vi "NEO Swerve Drive.vi"(7 "Operation":T4, 9 "Drive Conditions":T3, 10 "Robot Velocities":T9, 11 "Motors In":T5 {"Steer Scaling" format="%.2f"; "Drive Scaling" format="%.2f"; "Pod Locations (ft)"."Right Back Position" format="%.2f"; "Pod Locations (ft)"."Right Front Position" format="%.2f"; "Pod Locations (ft)"."Left Back Position" format="%.2f"; "Pod Locations (ft)"."Left Front Position" format="%.2f"}) -> (0 "Arbitrary":T1, 3 "Pod Setpoints (ft/s and deg)":T8)   [LabVIEW 2023]
uses:
  Type Definitions/Data/Pod Setpoints.ctl
  Type Definitions/Data/Pod Positions.ctl
  Type Definitions/Hardware/Swerve Drives/(NEO-NEO-ThroughBore-Pigeon2) Swerve.ctl
  Drive/Implementation/Drive Operations.ctl
  Type Definitions/Data/Robot Velocities.ctl
  Drive Conditions.ctl
  <vilib>/REV Custom Controls/REVSparkRefnum.ctl
  <vilib>/REVLibDriver/REVLibDriver.lvlib
panel:
  out "Waveform Chart":T2(graph)
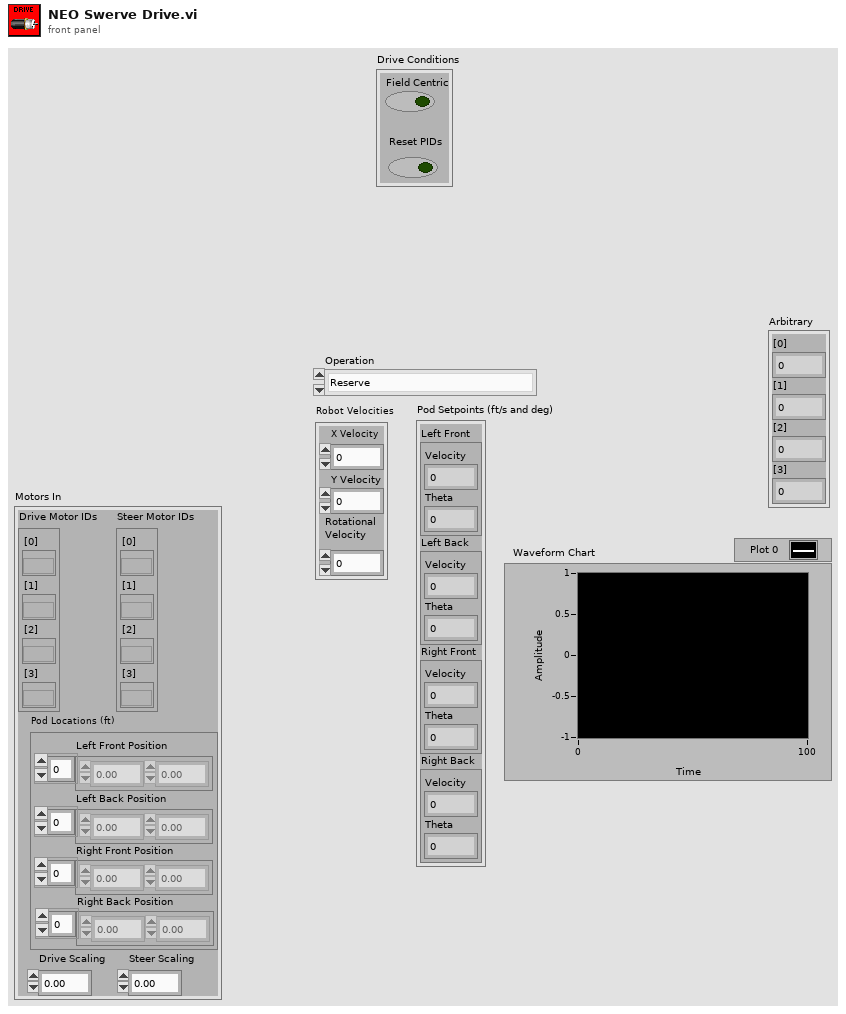
[diagram p1: front panel]
types:
  T1 = cluster{"[0]":dbl, "[1]":dbl, "[2]":dbl, "[3]":dbl}
  T2 = cluster{"Left Front":dbl, "Left Back":dbl, "Right Front":dbl, "Right Back":dbl}
  T3 = typedef "Drive Conditions.ctl" = cluster{"Field Centric":bool, "Reset PIDs":bool}
  T4 = typedef "Drive Operations.ctl" = enum16{"Reserve", "Read Current", "Immediate", "Calibrate", "Auto", "Auto Pickup"}
  T5 = typedef "(NEO-NEO-ThroughBore-Pigeon2) Swerve.ctl" = cluster{"Drive Motor IDs":cluster{"[0]":T6, "[1]":T6, "[2]":T6, "[3]":T6}, "Steer Motor IDs":cluster{"[0]":T6, "[1]":T6, "[2]":T6, "[3]":T6}, "Pod Locations (ft)":T7, "Drive Scaling":dbl, "Steer Scaling":dbl}
  T6 = typedef "REVLibDriver.lvlib/REVSparkRefnum.ctl" = refnum<k20>
  T7 = typedef "Pod Positions.ctl" = cluster{"Left Front Position":dbl[], "Left Back Position":dbl[], "Right Front Position":dbl[], "Right Back Position":dbl[]}
  T8 = typedef "Pod Setpoints.ctl" = cluster{"Left Front":cluster{"Velocity":dbl, "Theta":dbl}, "Left Back":cluster{"Velocity":dbl, "Theta":dbl}, "Right Front":cluster{"Velocity":dbl, "Theta":dbl}, "Right Back":cluster{"Velocity":dbl, "Theta":dbl}}
  T9 = typedef "Robot Velocities.ctl" = cluster{"X Velocity":dbl, "Y Velocity":dbl, "Rotational \nVelocity":dbl}
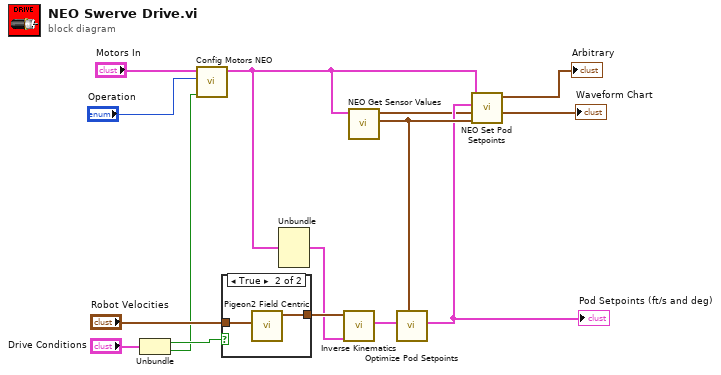
[diagram p0: block diagram]
diagram:
  n1 = Unbundle("Drive Conditions") -> ("Field Centric"=w6:bool, "Reset PIDs"=w2:bool)
  n2 = call "Config Motors NEO.vi"("Reset PIDs"=w2, "Operation"="Operation", "Motors In"="Motors In") -> ("Motors Out"=w11:T5)  [unwired: 8 in]
  n3 = case shown="True" w6 {
    tunnel: "Robot Velocities" -> [w15 w17]
    tunnel: [w15 w16] -> w3
    frame False {
    }
    frame True {
      n4 = call "Pigeon2 Field Centric.vi"("Field Centric Velocities"=w17) -> ("Robot Centric Velocities"=w16:T9)  [unwired: 10 in]
    }
  }
  n5 = Unbundle(w11) -> ("Pod Locations (ft)"=w1:T7)  [unwired: 4 out]
  n6 = call "Inverse Kinematics.vi"("Radii (ft)"=w1, "Target Velocity (ft/s and deg/s)"=w3) -> ("Pod Setpoints (ft/s and deg)"=w9:T8)  [unwired: 7 in, 2 out]
  n7 = call "NEO Get Sensor Values.vi"("Motors In"=w11) -> ("Steer Angles (degrees)"=w13:T2, "Drive Velocities (ft/s)"=w5:T2)  [unwired: 9 in]
  "Waveform Chart" <- w5
  n8 = call "Optimize Pod Setpoints.vi"("Current Pod Steering (deg)"=w13, "Initial Pod Setpoints (ft/s and deg)"=w9) -> ("Optimized Pod Setpoints (ft/s and deg)"=w8:T8)  [unwired: 9 in]
  "Pod Setpoints (ft/s and deg)" <- w8
  n9 = call "NEO Set Pod Setpoints.vi"("Steer Angles (degrees)"=w13, "Drive Velocities (ft/s)"=w5, "Pod Setpoints (ft/s and deg)"=w8, "Motors In"=w11) -> ("Arbitrary"=→"Arbitrary":T1)  [unwired: 7 in]
